vi "fpzoo.vi"() -> ()   [LabVIEW 2020]
uses:
  <vilib>/functionblocks/FB Property/FB Overlay U8.ctl
  <vilib>/functionblocks/FB Property/FB Overlay I8.ctl
  <vilib>/functionblocks/FB Property/FB Overlay I16.ctl
  <vilib>/functionblocks/FB Property/FB Overlay I32.ctl
  <vilib>/functionblocks/FB Property/FB Overlay I64.ctl
  <vilib>/functionblocks/FB Property/FB Overlay U16.ctl
  <vilib>/functionblocks/FB Property/FB Overlay U32.ctl
  <vilib>/functionblocks/FB Property/FB Overlay U64.ctl
  <vilib>/functionblocks/FB Property/FB Overlay SGL.ctl
  <vilib>/functionblocks/FB Property/FB Overlay String.ctl
  <vilib>/functionblocks/FB Property/FB Overlay Bool.ctl
  <vilib>/Array/Bytestream/Datum.ctl
  <vilib>/Array/Bytestream/Bytestream.lvclass
panel:
  in  "ErrIn":errorcluster
  in  "DatumCtl":T1
  in  "BoolRepCtl":T2 items=["FALSE", "TRUE"]
  in  "StrRepCtl":T3
  in  "SGLCtl":T4
  in  "U64Ctl":T5
  in  "U32Ctl":T6
  in  "U16Ctl":T7
  in  "I64Ctl":T8
  in  "I32Ctl":T9
  in  "I16Ctl":T10
  in  "I8Ctl":T11
  in  "U8Ctl":T12
  out "BoolOut":bool
  in  "BoolIn":bool
  out "StrOut":string
  in  "StrIn":string
  out "NumOut":dbl
  in  "NumIn":dbl
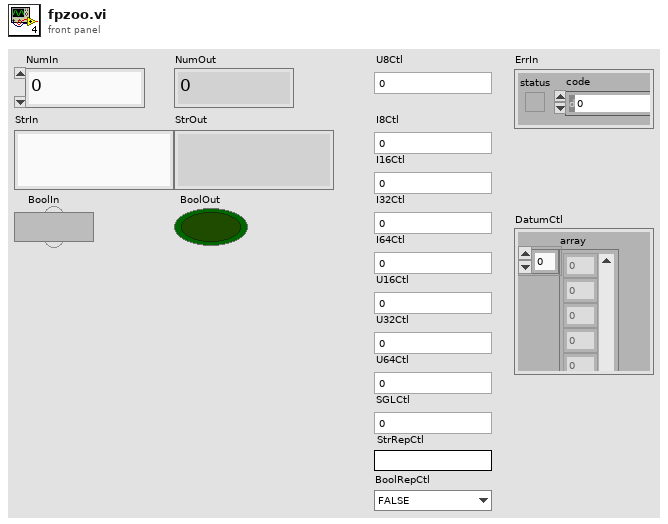
[diagram p1: front panel]
types:
  T1 = typedef "NI_Bytestream.lvlib/Bytestream.lvclass/Datum.ctl" = cluster{"array":u8[], "index":i32}
  T2 = typedef "FB Overlay Bool.ctl" = u16
  T3 = typedef "FB Overlay String.ctl" = string
  T4 = typedef "FB Overlay SGL.ctl" = sgl
  T5 = typedef "FB Overlay U64.ctl" = u64
  T6 = typedef "FB Overlay U32.ctl" = u32
  T7 = typedef "FB Overlay U16.ctl" = u16
  T8 = typedef "FB Overlay I64.ctl" = i64
  T9 = typedef "FB Overlay I32.ctl" = i32
  T10 = typedef "FB Overlay I16.ctl" = i16
  T11 = typedef "FB Overlay I8.ctl" = i8
  T12 = typedef "FB Overlay U8.ctl" = u8
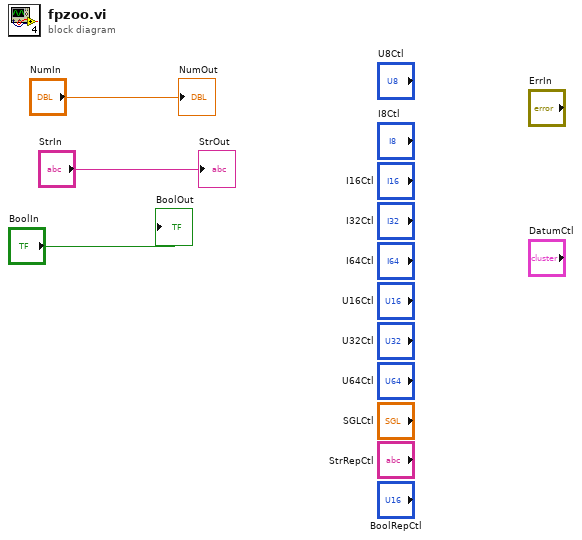
[diagram p0: block diagram]
diagram:
  "NumOut" <- "NumIn"
  "StrOut" <- "StrIn"
  "BoolOut" <- "BoolIn"
